vi "calculate_strain_from_array_normalized3__8910ab378b.vi"(7 "real strain":dbl[](array[numeric]), 9 "Gap":dbl, 10 "voltage to displacement contant":dbl, 11 "initial position in voltage":dbl) -> (2 "real strain (-)":dbl[](array[numeric]))   [LabVIEW 2023]
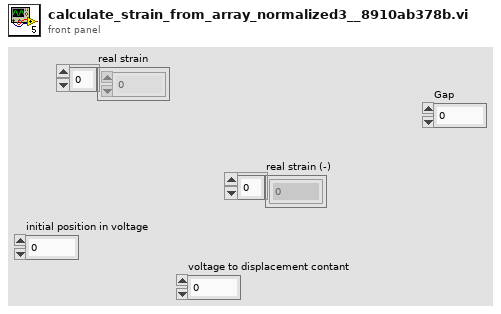
[diagram p1: front panel]
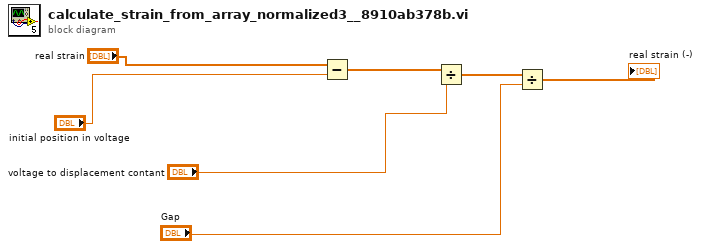
[diagram p0: block diagram]
diagram:
  n1 = Subtract(x="real strain", y="initial position in voltage") -> (x-y=w5:dbl[])
  n2 = Divide(x=w5, y="voltage to displacement contant") -> (x/y=w6:dbl[])
  n3 = Divide(x=w6, y="Gap") -> (x/y=→"real strain (-)":dbl[])
